vi "PathPlanner_Trajectory_GenerateStates_Pass3.vi"(9 "StartingSpeeds":T1 {"vOmega" format="%10.3f"; "vY" format="%10.3f"; "vX" format="%10.3f"}, 11 "in PathPlannerStates":T2[](array[typedef]) {"TargetHolonomicRotation"."SIN" format="%13.4f"; "TargetHolonomicRotation"."COS" format="%13.4f"; "TargetHolonomicRotation"."VALUE" format="%13.4f"; "Heading"."SIN" format="%13.4f"; "Heading"."COS" format="%13.4f"; "Heading"."VALUE" format="%13.4f"; "PositionMeters"."Y" format="%14.3f"; "PositionMeters"."X" format="%14.3f"}) -> (3 "out PathPlannerStates":T2[](array[typedef]) {"TargetHolonomicRotation"."SIN" format="%13.4f"; "TargetHolonomicRotation"."COS" format="%13.4f"; "TargetHolonomicRotation"."VALUE" format="%13.4f"; "Heading"."SIN" format="%13.4f"; "Heading"."COS" format="%13.4f"; "Heading"."VALUE" format="%13.4f"; "PositionMeters"."Y" format="%14.3f"; "PositionMeters"."X" format="%14.3f"})   [LabVIEW 2019, in "PathPlanner24.lvlib"]
doc: "Internal routine to help create a trajectory from a path."
uses:
  PathPlanner24.lvlib
  TypeDef/PathPlannerTrajectoryState.ctl
  <vilib>/Rock Robotics/WPI/ThirdParty/JAS_Junk/TrajLib/TypeDef/TRANSLATION2D.ctl
  <vilib>/Rock Robotics/WPI/ThirdParty/JAS_Junk/TrajLib/TypeDef/ROTATION2D.ctl
  TypeDef/PathPlannerPathConstraints.ctl
  <vilib>/Rock Robotics/WPI/ThirdParty/JAS_Junk/TrajLib/TypeDef/CHASSIS_SPEEDS.ctl
  <vilib>/Rock Robotics/WPI/ThirdParty/JAS_Junk/TrajLib/Rotation2d_UnaryMinus.vi
  <vilib>/Rock Robotics/WPI/ThirdParty/JAS_Junk/TrajLib/Rotation2d_RotateBy.vi
  <vilib>/Rock Robotics/WPI/ThirdParty/JAS_Junk/TrajLib/Rotation2d_CreateAngle.vi
  <vilib>/Rock Robotics/WPI/ThirdParty/JAS_Junk/TrajLib/Rotation2d_CreateXY.vi
  <vilib>/Rock Robotics/WPI/ThirdParty/JAS_Junk/TrajLib/Util_CalcDist.vi
  <vilib>/Rock Robotics/WPI/ThirdParty/JAS_Junk/TrajLib/Trajectory_Library.lvlib
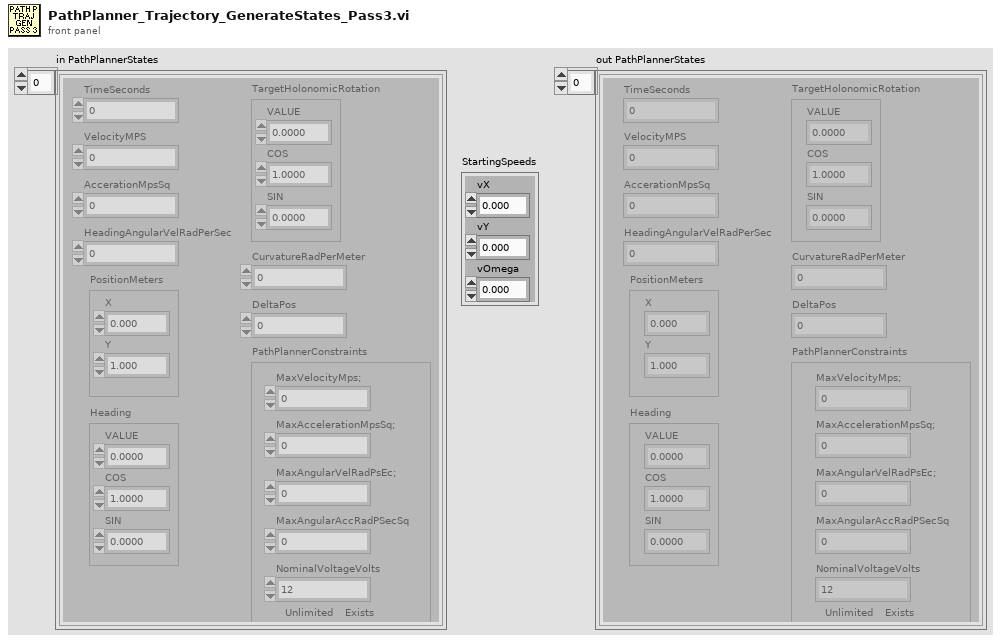
[diagram p1: front panel]
types:
  T1 = typedef "Trajectory_Library.lvlib/CHASSIS_SPEEDS.ctl" = cluster{"vX":dbl, "vY":dbl, "vOmega":dbl}
  T2 = typedef "PathPlanner24.lvlib/PathPlannerTrajectoryState.ctl" = cluster{"TimeSeconds":dbl, "VelocityMPS":dbl, "AccerationMpsSq":dbl, "HeadingAngularVelRadPerSec":dbl, "PositionMeters":T3, "Heading":T4, "TargetHolonomicRotation":T4, "CurvatureRadPerMeter":dbl, "PathPlannerConstraints":T5, "DeltaPos":dbl}
  T3 = typedef "Trajectory_Library.lvlib/TRANSLATION2D.ctl" = cluster{"X":dbl, "Y":dbl}
  T4 = typedef "Trajectory_Library.lvlib/ROTATION2D.ctl" = cluster{"VALUE":dbl, "COS":dbl, "SIN":dbl}
  T5 = typedef "PathPlanner24.lvlib/PathPlannerPathConstraints.ctl" = cluster{"MaxVelocityMps;":dbl, "MaxAccelerationMpsSq;":dbl, "MaxAngularVelRadPsEc;":dbl, "MaxAngularAccRadPSecSq":dbl, "Exists":bool, "Unlimited":bool, "NominalVoltageVolts":dbl}
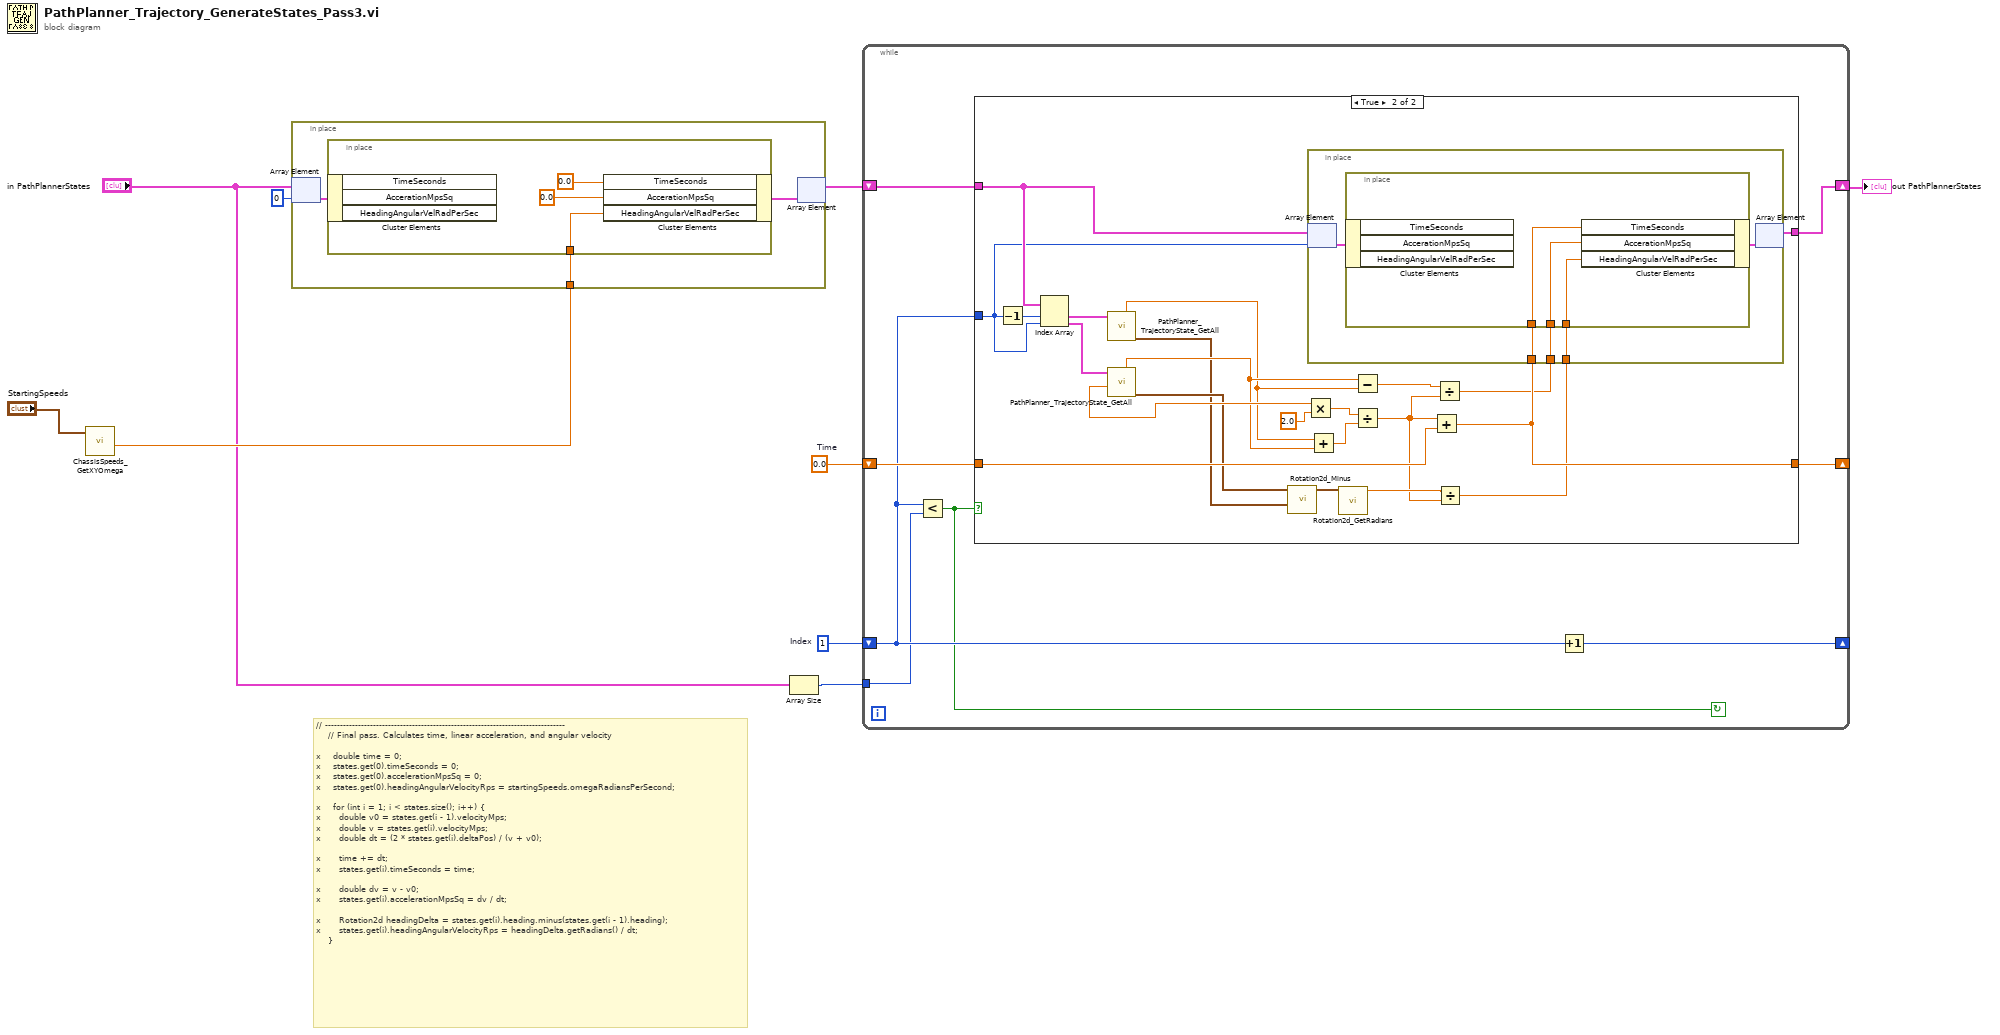
[diagram p0: block diagram]
diagram:
  w5 = 1  # Index
  w2 = 0.0  # Time
  # "// --------------------------------------------------------------------------------\n    // Final pass. Calculates time, linear acceleration, and angular velocity\n\nx    double time = 0;\nx    states.get(0).timeSeconds = 0;\nx    states.get(0).accelerationMpsSq = 0;\nx    states.get(0).headingAngularVelocityRps = startingSpeeds.omegaRadiansPerSecond;\n\nx    for (int i = 1; i < states.size(); i++) {\nx      double v0 = states.get(i - 1).velocityMps;\nx      double v = states.get(i).velocityMps;\nx      double dt = (2 * states.get(i).deltaPos) / (v + v0);\n\nx      time += dt;\nx      states.get(i).timeSeconds = time;\n\nx      double dv = v - v0;\nx      states.get(i).accelerationMpsSq = dv / dt;\n\nx      Rotation2d headingDelta = states.get(i).heading.minus(states.get(i - 1).heading);\nx      states.get(i).headingAngularVelocityRps = headingDelta.getRadians() / dt;\n    }"
  n1 = call <vilib>:"ChassisSpeeds_GetXYOmega.vi"("CHASSIS"="StartingSpeeds") -> ("vAngular"=w7:dbl)  [unwired: 8 in, 2 out]
  n2 = in-place {
    in-place-border: w7 -> [w10]
    n3 = in-place-array #1("in PathPlannerStates", 0) -> (w12:T2)
    n4 = in-place {
      in-place-border: w10 -> [w13]
      n5 = in-place-cluster #2(w12) -> ()  [unwired: 3 out]
      n6 = in-place-cluster #2("TimeSeconds"=0.0, "AccerationMpsSq"=0.0, "HeadingAngularVelRadPerSec"=w13) -> (w11:T2)
    }
    n7 = in-place-array #1(w11) -> (w6:T2[])  [unwired: 1 out]
  }
  n8 = Array Size(array="in PathPlannerStates") -> (size(s)=w3:i32)
  n9 = while {
    shift-right: [w22] -> w1
    shift-left: w6 -> [w21]
    shift-right: [w23] -> _
    shift-left: w5 -> [w18]
    tunnel: w3 -> [w17]
    shift-right: [w19] -> _
    shift-left: w2 -> [w20]
    stop <- w16 continue-if-true
    n10 = Less?(x=w18, y=w17) -> (x < y?=w16:bool)
    n11 = case shown="True" w16 {
      tunnel: [w25 w47] -> w22
      tunnel: w21 -> [w25 w45]
      tunnel: w20 -> [w24 w38]
      tunnel: [w24 w37] -> w19
      tunnel: w18 -> [_ w26]
      frame False {
      }
      frame True {
        n12 = Decrement(x=w26) -> (x-1=w46:i32)
        n13 = Index Array(array=w45, index #1=w46, index #2=w26) -> (element #1=w44:T2, element #2=w43:T2)
        n14 = call "PathPlanner_TrajectoryState_GetAll.vi"("PathPlannerState"=w44) -> ("Heading"=w31:T4, "VelocityMPS"=w35:dbl)  [unwired: 1 in, 8 out]
        n15 = call "PathPlanner_TrajectoryState_GetAll.vi"("PathPlannerState"=w43) -> ("Heading"=w32:T4, "VelocityMPS"=w36:dbl, "DeltaPos"=w41:dbl)  [unwired: 1 in, 7 out]
        n16 = call <vilib>:"Rotation2d_Minus.vi"("other ROTATION"=w31, "in ROTATION"=w32) -> ("out ROTATION"=w30:T4)  [unwired: 9 in]
        n17 = Multiply(x=w41, y=2.0) -> (x*y=w40:dbl)
        n18 = Add(x=w35, y=w36) -> (x+y=w39:dbl)
        n19 = call <vilib>:"Rotation2d_GetRadians.vi"("in ROTATION"=w30) -> ("AngleRadians"=w29:dbl)  [unwired: 10 in]
        n20 = Subtract(x=w36, y=w35) -> (x-y=w34:dbl)
        n21 = Divide(x=w40, y=w39) -> (x/y=w28:dbl)
        n22 = Add(x=w28, y=w38) -> (x+y=w37:dbl)
        n23 = Divide(x=w34, y=w28) -> (x/y=w33:dbl)
        n24 = Divide(x=w29, y=w28) -> (x/y=w27:dbl)
        n25 = in-place {
          in-place-border: w37 -> [w50]
          in-place-border: w33 -> [w49]
          in-place-border: w27 -> [w48]
          n26 = in-place-array #3(w45, w26) -> (w52:T2)
          n27 = in-place {
            in-place-border: w50 -> [w55]
            in-place-border: w49 -> [w54]
            in-place-border: w48 -> [w53]
            n28 = in-place-cluster #4(w52) -> ()  [unwired: 3 out]
            n29 = in-place-cluster #4("TimeSeconds"=w55, "AccerationMpsSq"=w54, "HeadingAngularVelRadPerSec"=w53) -> (w51:T2)
          }
          n30 = in-place-array #3(w51) -> (w47:T2[])  [unwired: 1 out]
        }
      }
    }
    n31 = Increment(x=w18) -> (x+1=w23:i32)
  }
  "out PathPlannerStates" <- w1
